vi "DUT_Commands_List.vi"(7 "PCB Serial No":string, 8 "error in":errorcluster, 9 "DUT Cmd":T2=enum."Stop console logs", 10 "Operation":T1=enum."write&Read", 11 "Resource In":refnum<visa-resource-name>) -> (0 "error out":errorcluster, 2 "Command Response":string, 3 "Resource out":refnum<visa-resource-name>)   [LabVIEW 2021]
uses:
  DUT_Cmd.ctl
  10054_Control Folder/Support/Relay_no.ctl
panel:
  in  "Password":string
  in  "SSID":string
  out "read buffer":string
  out "Write":string
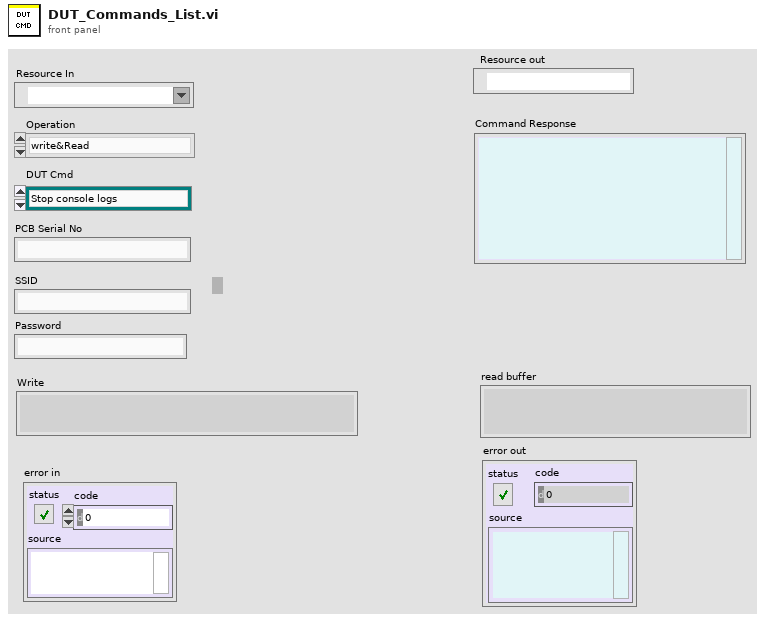
[diagram p1: front panel]
types:
  T1 = typedef "Relay_no.ctl" = enum16{"Init", "write&Read", "PCB Serial Write & Read", "PCB Write SSD & Password", "Read Wifi state", "Reset", "Close"}
  T2 = typedef "DUT_Cmd.ctl" = enum16{"Unlock serial", "Stop console logs", "Release emergency at start", "Read firmware", "WiFi credentials", "WiFi connected", "WiFi SSID", "Board revision", "ADC_NTC_TEMP", "ADC_TYPE2_RCD_CURRENT", "PCBA serial write", "PCBA serial readback", "Start energy meter", "Energy meter Vac", "Energy meter Iac", "Energy meter PF", "Energy meter energy", "Provision", "Set gateway identity", "CP checklist", "Earth detect", "D+M sense unplugged", "D+M sense plugged", "Output relay weld", "Start diagnostics", "Relay 1 on", "Relay 2 on", "Emergency pressed", "Release emergency", "Emergency released", "Unlock serial for 5 A", "Board current (5 A)", "Unlock serial for 15 A", "Board current (15 A)", "Unlock serial for 0 A", "NFC tag", "Start diagnostics again", "Relay 2 off", "Relay 1 off", "End diagnostics", "Load current (5 A) [No USB station]", "Load current (15 A) [No USB station]", "Load current (0 A) [No USB station]", "NFC tag [No USB station]", "Battery Voltage", "FW Power reset", "Notification LED", "O/P Relay weld Detection", "Earth Detection", "12V ", "5V", "3.3V"}
  T3 = cluster{"baud rate":u32, "data bits":u16, "parity":enum16{"None", "Odd", "Even", "Mark", "Space"}, "stop bits":u16, "flow control":u16}
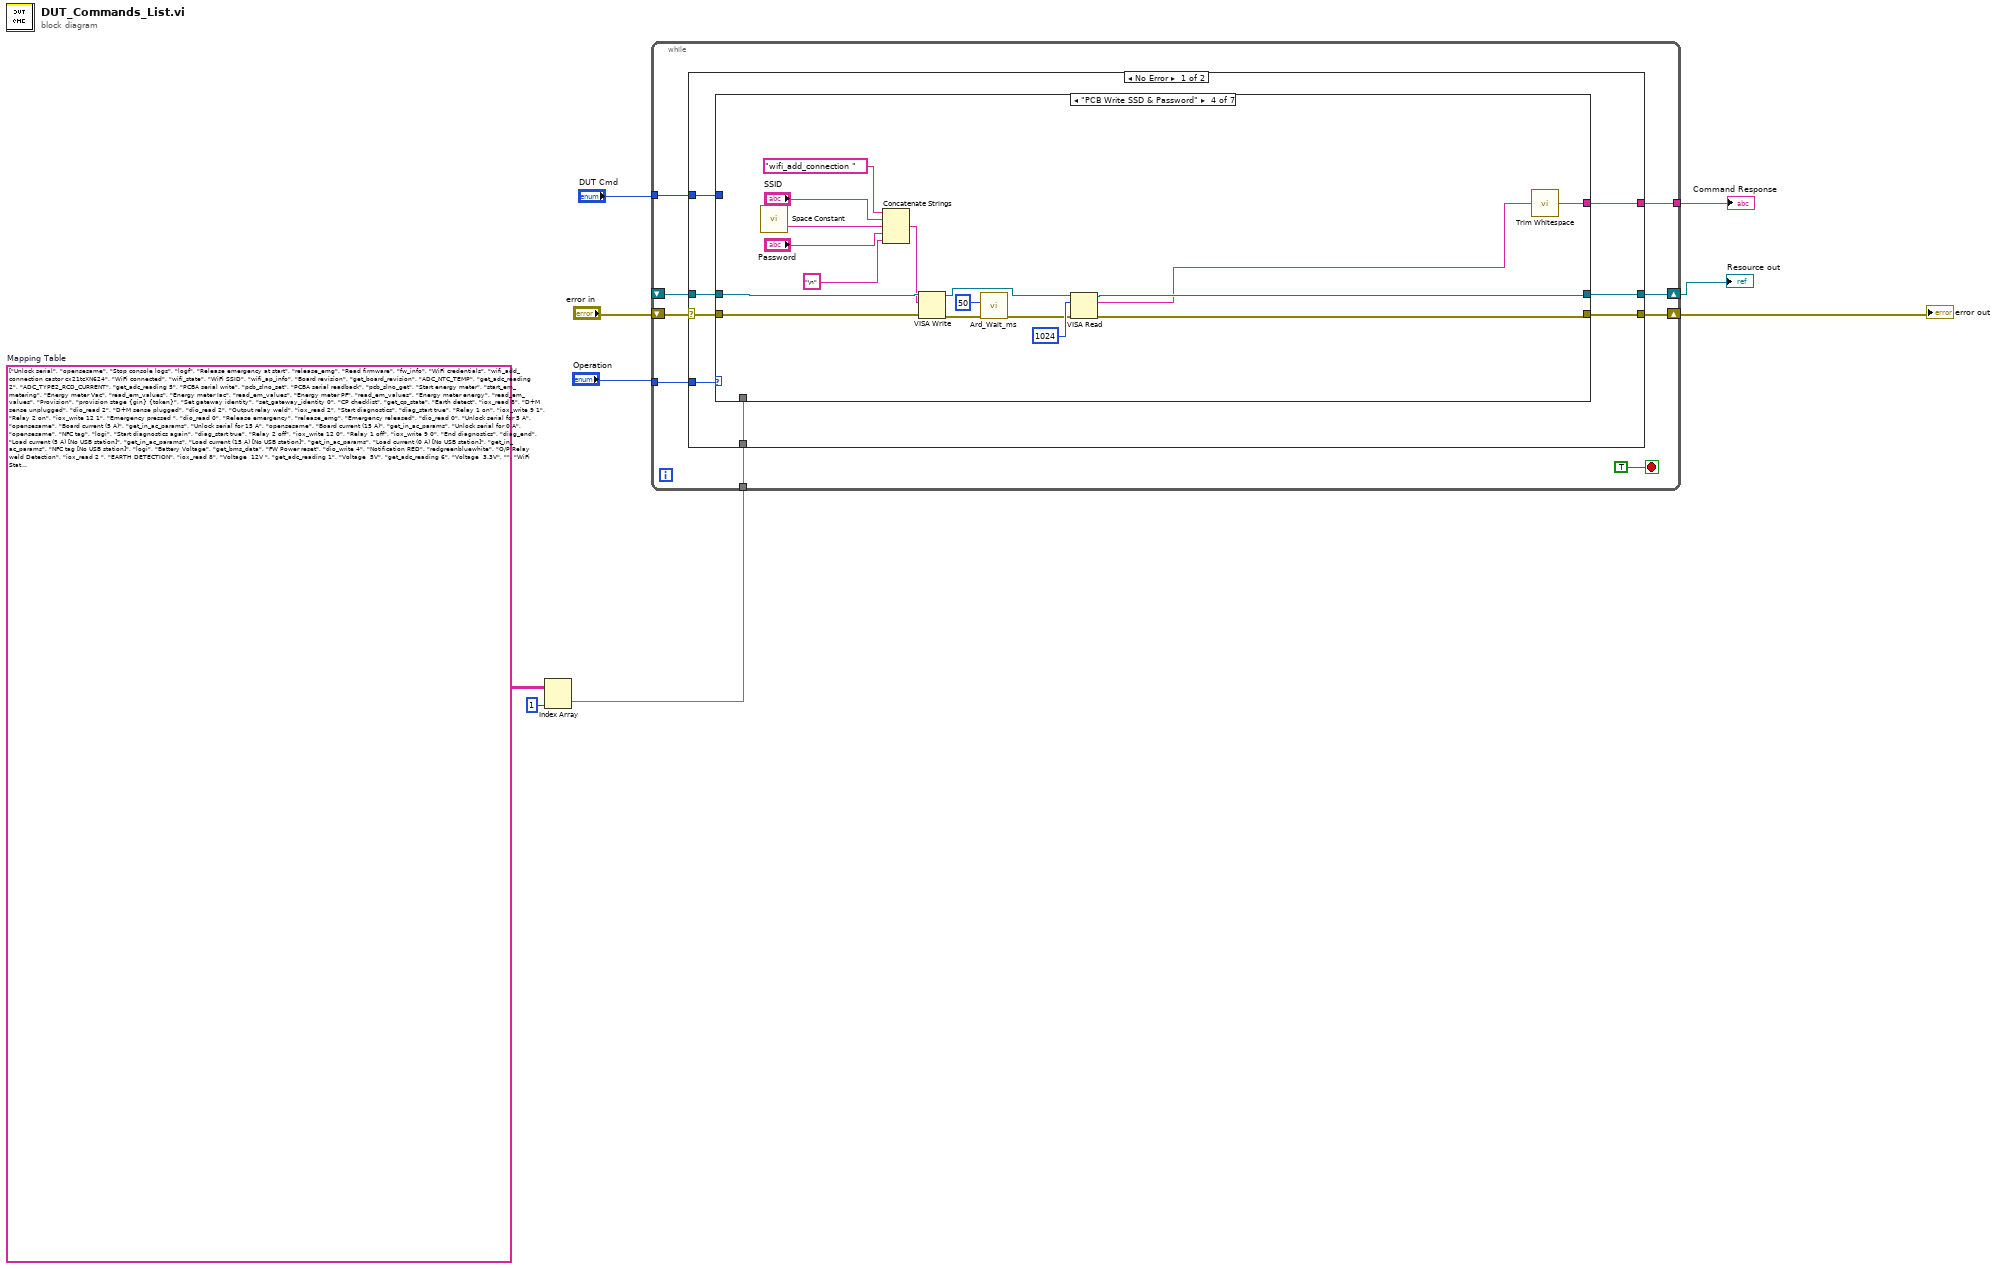
[diagram p0: block diagram]
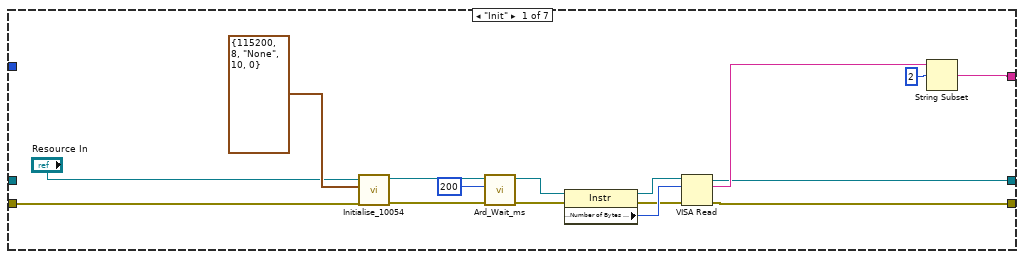
[diagram p2: hidden frame]
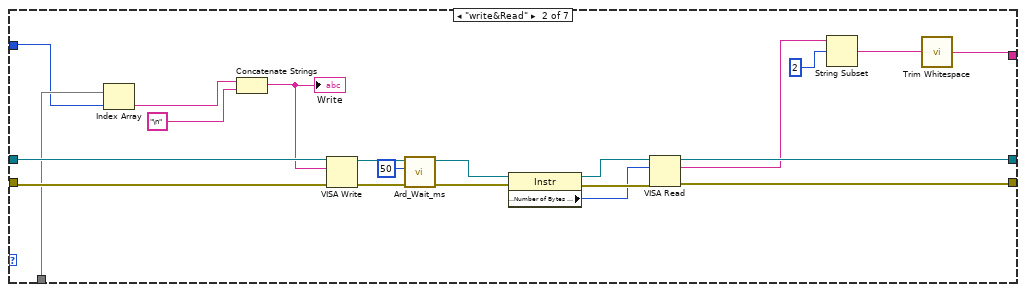
[diagram p3: hidden frame]
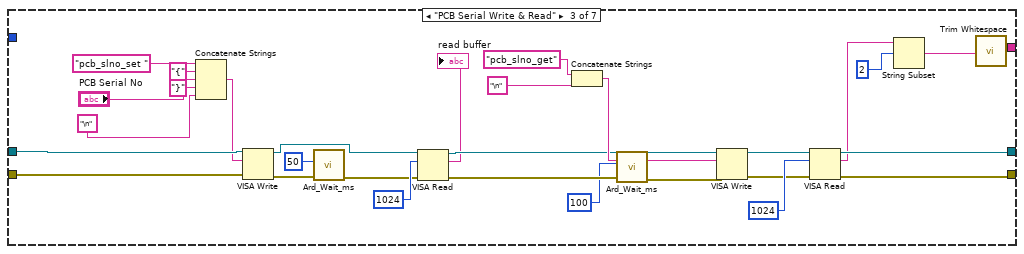
[diagram p4: hidden frame]
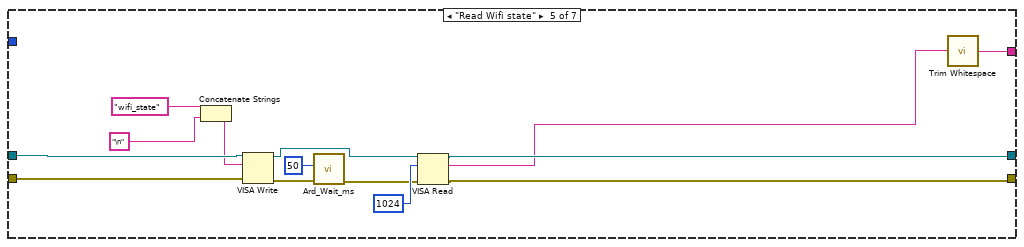
[diagram p5: hidden frame]
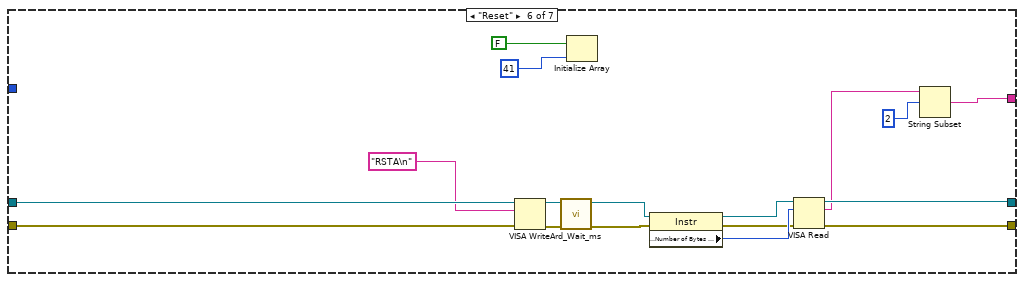
[diagram p6: hidden frame]
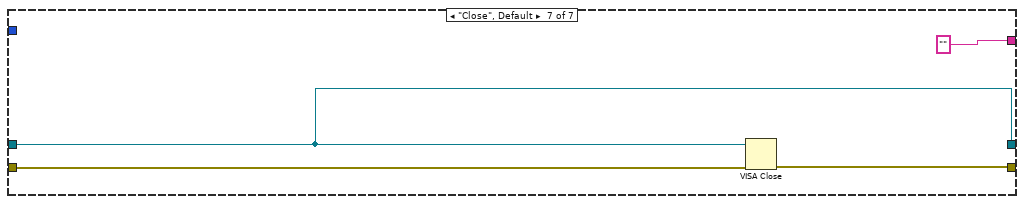
[diagram p7: hidden frame]
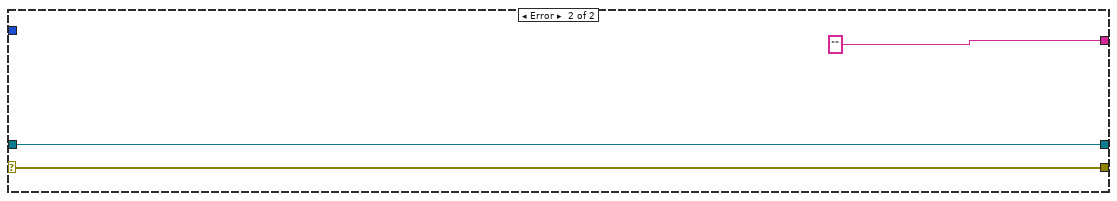
[diagram p8: hidden frame]
diagram:
  w6 = string[][] [["Unlock serial", "opensesame"], ["Stop console logs", "logf"], ["Release emergency at start", "release_emg"], ["Read firmware", "fw_info"], ["WiFi credentials", "wifi_add_connection castor cx21tcXN624"], ["WiFi connected", "wifi_state"], ["WiFi SSID", "wifi_ap_info"], ["Board revision", "get_board_revision"], ["ADC_NTC_TEMP", "get_adc_reading 2"], ["ADC_TYPE2_RCD_CURRENT", "get_adc_reading 5"], ["PCBA serial write", "pcb_slno_set"], ["PCBA serial readback", "pcb_slno_get"], ["Start energy meter", "start_em_metering"], ["Energy meter Vac", "read_em_values"], ["Energy meter Iac", "read_em_values"], ["Energy meter PF", "read_em_values"], ["Energy meter energy", "read_em_values"], ["Provision", "provision stage {gin} {token}"], ["Set gateway identity", "set_gateway_identity 0"], ["CP checklist", "get_cp_state"], ["Earth detect", "iox_read 8"], ["D+M sense unplugged", "dio_read 2"], ["D+M sense plugged", "dio_read 2"], ["Output relay weld", "iox_read 2"], ["Start diagnostics", "diag_start true"], ["Relay 1 on", "iox_write 9 1"], ["Relay 2 on", "iox_write 12 1"], ["Emergency pressed ", "dio_read 0"], ["Release emergency", "release_emg"], ["Emergency released", "dio_read 0"], ["Unlock serial for 5 A", "opensesame"], ["Board current (5 A)", "get_in_ac_params"], ["Unlock serial for 15 A", "opensesame"], ["Board current (15 A)", "get_in_ac_params"], ["Unlock serial for 0 A", "opensesame"], ["NFC tag", "logi"], ["Start diagnostics again", "diag_start true"], ["Relay 2 off", "iox_write 12 0"], ["Relay 1 off", "iox_write 9 0"], ["End diagnostics", "diag_end"], ["Load current (5 A) [No USB station]", "get_in_ac_params"], ["Load current (15 A) [No USB station]", "get_in_ac_params"], ["Load current (0 A) [No USB station]", "get_in_ac_params"], ["NFC tag [No USB station]", "logi"], ["Battery Voltage", "get_bms_data"], ["FW Power reset", "dio_write 4"], ["Notification RED", "redgreenbluewhite"], ["O/P Relay weld Detection", "iox_read 2 "], ["EARTH DETECTION", "iox_read 8"], ["Voltage  12V ", "get_adc_reading 1"], ["Voltage  5V", "get_adc_reading 6"], ["Voltage  3.3V", ""], ["WiFi State", "wifi_state"], ["WiFi SSID", "wifi_ap_info"]]  # Mapping Table
  n1 = Index Array(array=w6, index (col)=1 ("disabled index (col)")) -> (element=w4:string[])  [unwired: 1 in]
  n2 = while {
    tunnel: "Operation" -> [w17]
    shift-right: [w16] -> w7
    shift-left: _ -> [w14]
    shift-right: [w15] -> w1
    shift-left: "error in" -> [w13]
    tunnel: [w12] -> w8
    tunnel: "DUT Cmd" -> [w11]
    tunnel: w4 -> [w10]
    stop <- TRUE stop-if-true
    n3 = case shown="No Error" w13 {
      selector: w13 -> [w22 w143]
      tunnel: w17 -> [w26 _]
      tunnel: [w25 w145] -> w16
      tunnel: [w24 w143] -> w15
      tunnel: w14 -> [w23 w145]
      tunnel: [w21 "" ("read buffer")] -> w12
      tunnel: w11 -> [w20 _]
      tunnel: w10 -> [w19 _]
      frame No Error {
        n4 = case shown="\"PCB Write SSD & Password\"" w26 {
          tunnel: [w32 w57 w89 w95 w112 w133 w141] -> w25
          tunnel: w22 -> [w39 w50 w85 w106 w120 w126 w140]
          tunnel: [w30 w58 w90 w94 w111 w134 w139] -> w24
          tunnel: w23 -> [_ w61 w91 w108 w122 w138 w141]
          tunnel: [w31 w43 w82 w104 w118 w127 "" ("read buffer")] -> w21
          tunnel: w20 -> [_ w46 _ _ _ _ _]
          tunnel: w19 -> [_ w49 _ _ _ _ _]
          frame "Init" {
            n5 = call "Initialise_10054 .vi"("error in"=w39, "Serial Settings"=T3 {"baud rate"=115200, "data bits"=8, "parity"=enum."None", "stop bits"=10, "flow control"=0}, "RS232 name in"="Resource In") -> ("error out"=w28:errorcluster, "RS232 name out"=w27:refnum<visa-resource-name>)  [unwired: 7 in]
            n6 = call "Ard_Wait_ms.vi"("error in"=w28, "millisec"=u32 200) -> ("error in 2"=w35:errorcluster)  [unwired: 9 in]
            n7 = property class="Instr"(reference=w27, error in=w35) -> (reference out=w36:refnum<visa-resource-name>, error out=w37:errorcluster, "Serial Settings:Number of Bytes at Serial Port"=w38:u32)
            n8 = VISA Read(VISA resource name=w36, byte count=w38, error in (no error)=w37) -> (VISA resource name out=w32:refnum<visa-resource-name>, read buffer=w34:string, error out=w30:errorcluster)  [unwired: 1 out]
            n9 = String Subset(string=w34, offset (0)=2) -> (substring=w31:string)  [unwired: 1 in]
          }
          frame "write&Read" {
            n10 = Index Array(array=w49, index=w46) -> (element=w48:string)
            n11 = Concatenate Strings(w48, "\n") -> (w51:string)
            "Write" <- w51
            n12 = VISA Write(VISA resource name=w61, write buffer=w51, error in (no error)=w50) -> (VISA resource name out=w56:refnum<visa-resource-name>, error out=w55:errorcluster)  [unwired: 1 out]
            n13 = call "Ard_Wait_ms.vi"("error in"=w55, "millisec"=u32 50) -> ("error in 2"=w54:errorcluster)  [unwired: 9 in]
            n14 = property class="Instr"(reference=w56, error in=w54) -> (reference out=w59:refnum<visa-resource-name>, error out=w60:errorcluster, "Serial Settings:Number of Bytes at Serial Port"=w42:u32)
            n15 = VISA Read(VISA resource name=w59, byte count=w42, error in (no error)=w60) -> (VISA resource name out=w57:refnum<visa-resource-name>, read buffer=w53:string, error out=w58:errorcluster)  [unwired: 1 out]
            n16 = String Subset(string=w53, offset (0)=2) -> (substring=w44:string)  [unwired: 1 in]
            n17 = call <vilib>:"Trim Whitespace.vi"("string"=w44) -> ("trimmed string"=w43:string)  [unwired: 1 in]
          }
          frame "PCB Serial Write & Read" {
            n18 = Concatenate Strings("pcb_slno_set " ("string"), "{" ("string"), "PCB Serial No", "}" ("string"), "\n") -> (w86:string)
            n19 = VISA Write(VISA resource name=w91, write buffer=w86, error in (no error)=w85) -> (VISA resource name out=w65:refnum<visa-resource-name>, error out=w78:errorcluster)  [unwired: 1 out]
            n20 = call "Ard_Wait_ms.vi"("error in"=w78, "millisec"=u32 50) -> ("error in 2"=w64:errorcluster)  [unwired: 9 in]
            n21 = VISA Read(VISA resource name=w65, byte count=u32 1024, error in (no error)=w64) -> (VISA resource name out=w72:refnum<visa-resource-name>, read buffer=→"read buffer":string, error out=w70:errorcluster)  [unwired: 1 out]
            n22 = Concatenate Strings("pcb_slno_get" ("string"), "\n") -> (w75:string)
            n23 = call "Ard_Wait_ms.vi"("error in"=w70, "millisec"=u32 100) -> ("error in 2"=w69:errorcluster)  [unwired: 9 in]
            n24 = VISA Write(VISA resource name=w72, write buffer=w75, error in (no error)=w69) -> (VISA resource name out=w63:refnum<visa-resource-name>, error out=w62:errorcluster)  [unwired: 1 out]
            n25 = VISA Read(VISA resource name=w63, byte count=u32 1024, error in (no error)=w62) -> (VISA resource name out=w89:refnum<visa-resource-name>, read buffer=w88:string, error out=w90:errorcluster)  [unwired: 1 out]
            n26 = String Subset(string=w88, offset (0)=2) -> (substring=w83:string)  [unwired: 1 in]
            n27 = call <vilib>:"Trim Whitespace.vi"("string"=w83) -> ("trimmed string"=w82:string)  [unwired: 1 in]
          }
          frame "PCB Write SSD & Password" {
            n28 = call <vilib>:"Space Constant.vi"() -> ("String"=w92:string)
            n29 = Concatenate Strings("wifi_add_connection " ("string"), "SSID", w92, "Password", "\n") -> (w107:string)
            n30 = VISA Write(VISA resource name=w108, write buffer=w107, error in (no error)=w106) -> (VISA resource name out=w99:refnum<visa-resource-name>, error out=w101:errorcluster)  [unwired: 1 out]
            n31 = call "Ard_Wait_ms.vi"("error in"=w101, "millisec"=u32 50) -> ("error in 2"=w98:errorcluster)  [unwired: 9 in]
            n32 = VISA Read(VISA resource name=w99, byte count=u32 1024, error in (no error)=w98) -> (VISA resource name out=w95:refnum<visa-resource-name>, read buffer=w93:string, error out=w94:errorcluster)  [unwired: 1 out]
            n33 = call <vilib>:"Trim Whitespace.vi"("string"=w93) -> ("trimmed string"=w104:string)  [unwired: 1 in]
          }
          frame "Read Wifi state" {
            n34 = Concatenate Strings("wifi_state" ("string"), "\n") -> (w121:string)
            n35 = VISA Write(VISA resource name=w122, write buffer=w121, error in (no error)=w120) -> (VISA resource name out=w115:refnum<visa-resource-name>, error out=w117:errorcluster)  [unwired: 1 out]
            n36 = call "Ard_Wait_ms.vi"("error in"=w117, "millisec"=u32 50) -> ("error in 2"=w114:errorcluster)  [unwired: 9 in]
            n37 = VISA Read(VISA resource name=w115, byte count=u32 1024, error in (no error)=w114) -> (VISA resource name out=w112:refnum<visa-resource-name>, read buffer=w110:string, error out=w111:errorcluster)  [unwired: 1 out]
            n38 = call <vilib>:"Trim Whitespace.vi"("string"=w110) -> ("trimmed string"=w118:string)  [unwired: 1 in]
          }
          frame "Reset" {
            n39 = VISA Write(VISA resource name=w138, write buffer="RSTA\n", error in (no error)=w126) -> (VISA resource name out=w132:refnum<visa-resource-name>, error out=w131:errorcluster)  [unwired: 1 out]
            n40 = call "Ard_Wait_ms.vi"("error in"=w131) -> ("error in 2"=w130:errorcluster)  [unwired: 10 in]
            n41 = Initialize Array(FALSE, 41 ("dimension size")) -> ()  [unwired: 1 out]
            n42 = property class="Instr"(reference=w132, error in=w130) -> (reference out=w135:refnum<visa-resource-name>, error out=w136:errorcluster, "Serial Settings:Number of Bytes at Serial Port"=w137:u32)
            n43 = VISA Read(VISA resource name=w135, byte count=w137, error in (no error)=w136) -> (VISA resource name out=w133:refnum<visa-resource-name>, read buffer=w129:string, error out=w134:errorcluster)  [unwired: 1 out]
            n44 = String Subset(string=w129, offset (0)=2) -> (substring=w127:string)  [unwired: 1 in]
          }
          frame "Close", Default {
            n45 = VISA Close(VISA resource name=w141, error in (no error)=w140) -> (error out=w139:errorcluster)
          }
        }
      }
      frame Error {
      }
    }
  }
  "error out" <- w1
  "Command Response" <- w8
  "Resource out" <- w7
